vi "SaveCFG.vi"(7 "Clear Before Saving(F)":bool, 8 "error in (no error)":errorcluster, 11 "object in":refnum<class "Configuration.lvclass">) -> (0 "error out":errorcluster, 2 "OK?":bool, 3 "object out":refnum<class "Configuration.lvclass">)   [LabVIEW 2021, in "Channel.lvlib" / "Configuration.lvclass"]
doc: "Saves configuration"
uses:
  Configuration.lvclass
  Configuration.lvclass/Configuration.ctl
  <vilib>/Utility/config.llb/NI_LVConfig.lvlib
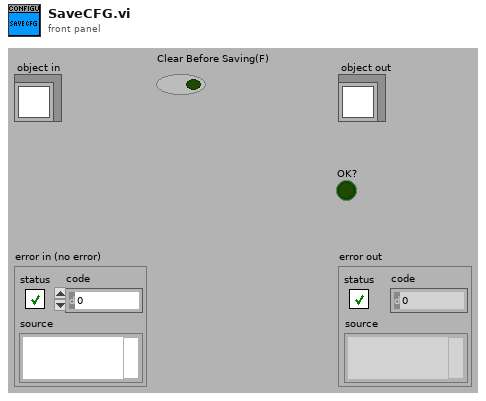
[diagram p1: front panel]
types:
  T1 = typedef "NI_LVConfig.lvlib/Config Data RefNum.ctl" = refnum<k1>
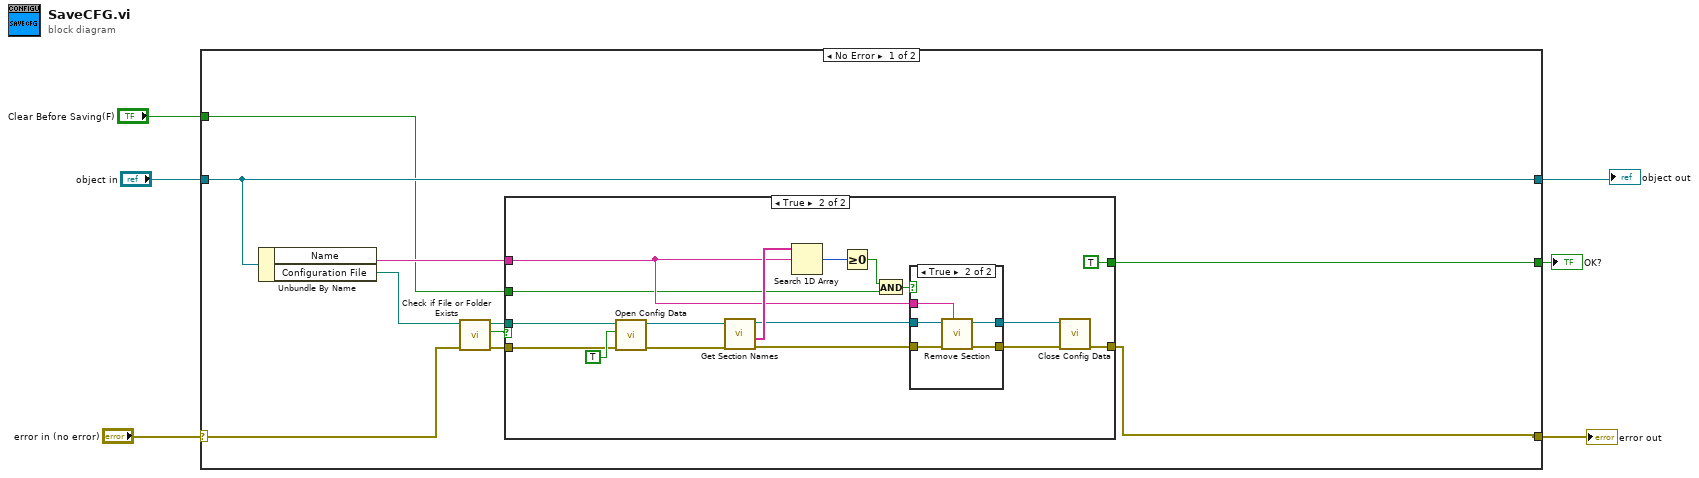
[diagram p0: block diagram]
diagram:
  n1 = case shown="No Error" "error in (no error)" {
    selector: "error in (no error)" -> [w13 w44]
    tunnel: [w8 w44] -> w3
    tunnel: [w16 w43] -> w6
    tunnel: "object in" -> [w16 w43]
    tunnel: [w10 _] -> w2
    tunnel: "Clear Before Saving(F)" -> [w7 _]
    frame No Error {
      n2 = Unbundle By Name(w16) -> ("Name"=w15:string, "Configuration File"=w14:path)
      n3 = call <vilib>:"Check if File or Folder Exists.vi"("error in (no error)"=w13, "path"=w14) -> ("error out"=w12:errorcluster, "file or folder exists?"=w11:bool, "dup path"=w9:path)  [unwired: 7 in]
      n4 = case shown="True" w11 {
        selector: w11 -> [w17 _]
        tunnel: [w18 w32] -> w8
        tunnel: w15 -> [_ w24]
        tunnel: w12 -> [w18 w31]
        tunnel: [w17 TRUE] -> w10
        tunnel: w9 -> [_ w30]
        tunnel: w7 -> [_ w20]
        frame False {
        }
        frame True {
          n5 = call <vilib>:"Open Config Data.vi"("error in (no error)"=w31, "create file if necessary (T)"=TRUE, "configuration file path"=w30) -> ("error out"=w33:errorcluster, "refnum"=w35:T1)  [unwired: 6 in, 1 out]
          n6 = call <vilib>:"Get Section Names.vi"("error in (no error)"=w33, "refnum"=w35) -> ("error out"=w26:errorcluster, "section names"=w29:string[], "refnum out"=w27:T1)  [unwired: 7 in]
          n7 = Search 1D Array(1D array=w29, element=w24) -> (index of element=w28:i32)  [unwired: 1 in]
          n8 = Greater Or Equal To 0?(x=w28) -> (x >= 0?=w22:bool)
          n9 = And(x=w22, y=w20) -> (x .and. y?=w21:bool)
          n10 = case shown="True" w21 {
            tunnel: w27 -> [w37 w42]
            tunnel: w26 -> [w36 w41]
            tunnel: [w37 w40] -> w25
            tunnel: w24 -> [_ w39]
            tunnel: [w36 w38] -> w23
            frame False {
            }
            frame True {
              n11 = call <vilib>:"Remove Section.vi"("section"=w39, "error in (no error)"=w41, "refnum"=w42) -> ("error out"=w38:errorcluster, "refnum out"=w40:T1)  [unwired: 6 in, 1 out]
            }
          }
          n12 = call <vilib>:"Close Config Data.vi"("error in (no error)"=w23, "refnum"=w25) -> ("error out"=w32:errorcluster)  [unwired: 8 in, 1 out]
        }
      }
    }
    frame Error {
    }
  }
  "error out" <- w3
  "object out" <- w6
  "OK?" <- w2
